vi "Day 9.vi"() -> ()   [LabVIEW 2021]
uses:
  e82450e5-71a3-46d6-8b92-650601a06453.vi
  <vilib>/Utility/file.llb/Read Delimited Spreadsheet (string).vi
  <vilib>/Comparison/Less/Less Functor/Less Functor.lvclass
panel:
  out "x-y":dbl
  out "Data":i32[][](array[numeric])
  out "Intensity Graph":i32[][](graph)
  out "Solution":i32
  in  "Input File":enum32{"example input", "input"}(radio)
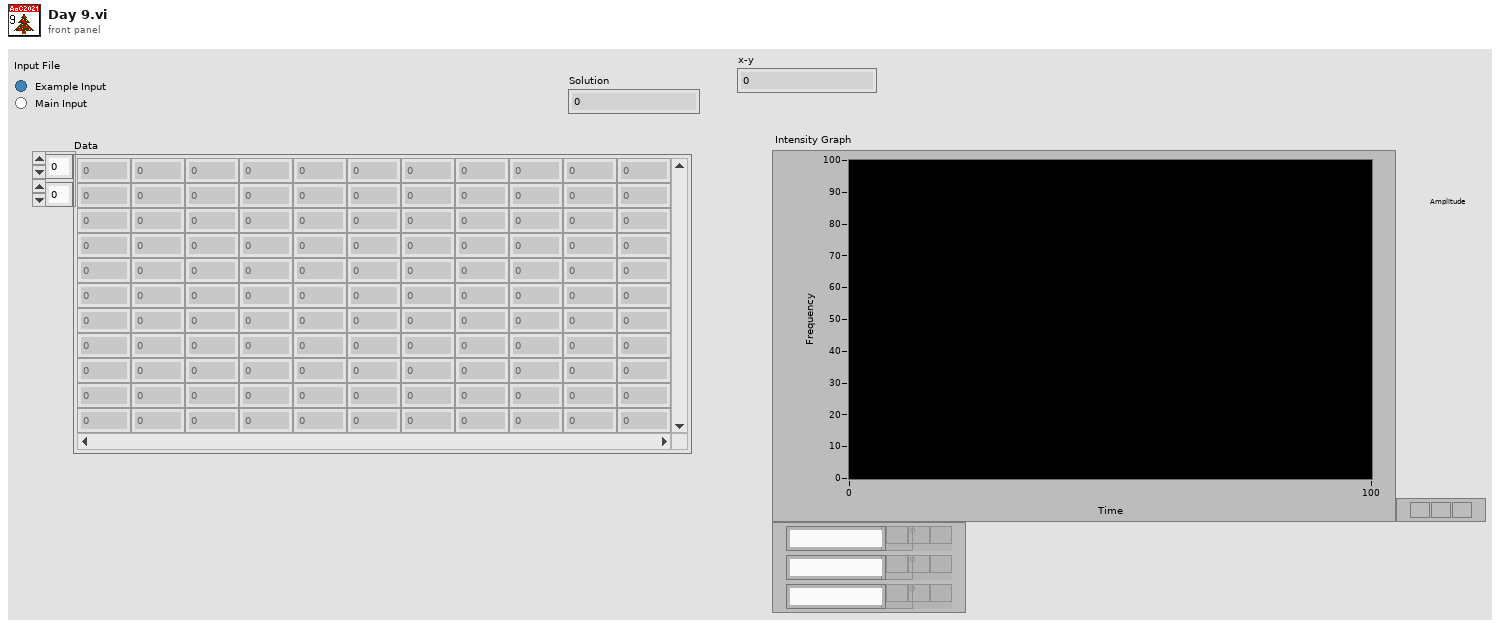
[diagram p1: front panel]
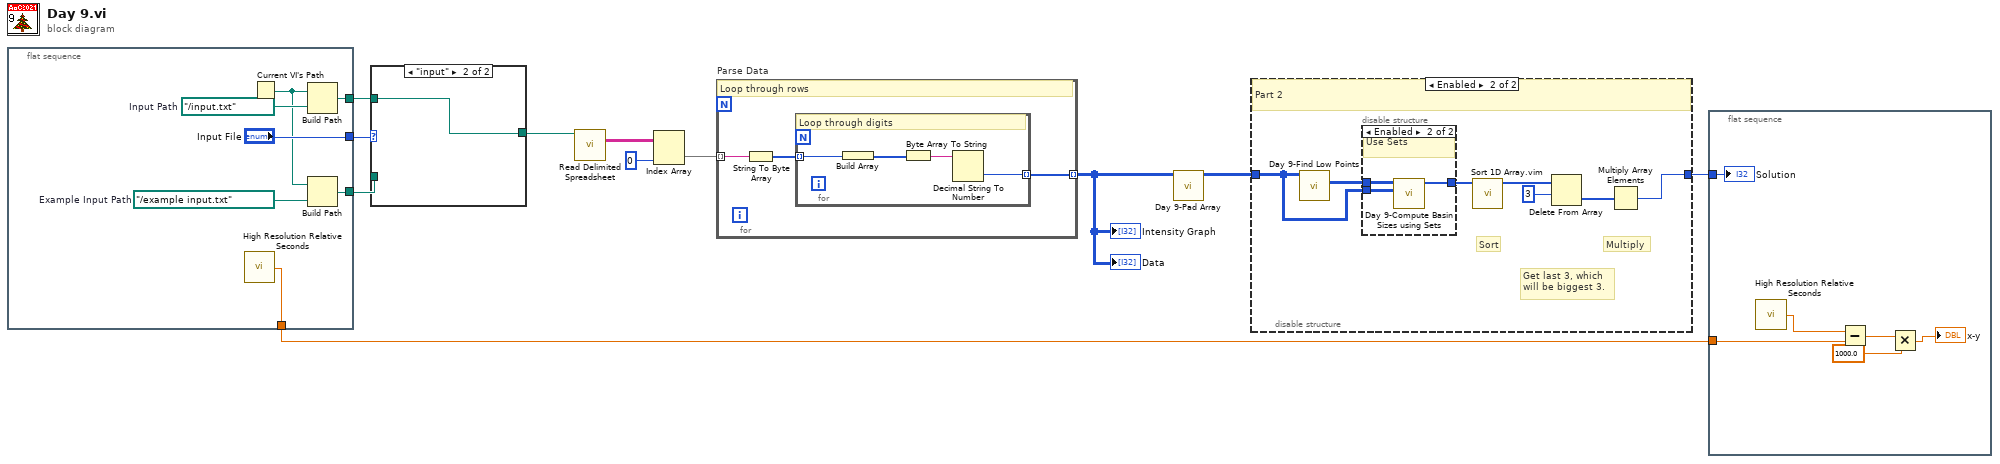
[diagram p0: block diagram]
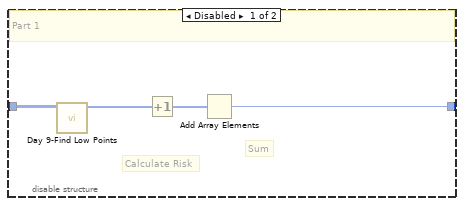
[diagram p3: hidden frame]
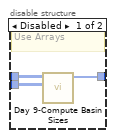
[diagram p4: hidden frame]
diagram:
  n1 = flat-sequence {
    tunnel: ["Input File"] -> w11
    tunnel: [w15] -> w10
    tunnel: [w14] -> w9
    tunnel: [w12] -> w1
    frame #0 {
      w17 = path "../example input.txt"  # Example Input Path
      w18 = path "../input.txt"  # Input Path
      n2 = call <vilib>:"High Resolution Relative Seconds.vi"() -> ("relative seconds"=w12:dbl)
      n3 = Current VI's Path() -> (path=w13:path)
      n4 = Build Path(base path=w13, name or relative path=w18) -> (appended path=w15:path)
      n5 = Build Path(base path=w13, name or relative path=w17) -> (appended path=w14:path)
    }
  }
  n6 = case shown="\"input\"" w11 {
    tunnel: w10 -> [_ w20]
    tunnel: w9 -> [w19 _]
    tunnel: [w19 w20] -> w8
    frame "example input" {
    }
    frame "input" {
    }
  }
  n7 = call-poly <vilib>:"Read Delimited Spreadsheet.vi"("file path (dialog if empty)"=w8) -> ("all rows"=w7:string[][])  [unwired: 9 in, 5 out]
  n8 = Index Array(array=w7, index (col)=0 ("disabled index (col)")) -> (element=w5:string[])  [unwired: 1 in]
  n9 = for "Parse Data" {
    tunnel: w5 -> [w23] mode=indexing
    tunnel: [w21] -> w3 mode=indexing
    # "Loop through rows"
    n10 = String To Byte Array(string=w23) -> (unsigned byte array=w22:u8[])
    n11 = for {
      tunnel: w22 -> [w27] mode=indexing
      tunnel: [w24] -> w21 mode=indexing
      # "Loop through digits"
      n12 = Build Array(w27) -> (w26:u8[])
      n13 = Byte Array To String(unsigned byte array=w26) -> (string=w25:string)
      n14 = Decimal String To Number(string=w25) -> (number=w24:i32)  [unwired: 2 in, 1 out]
    }
  }
  "Intensity Graph" <- w3
  "Data" <- w3
  n15 = call "Day 9-Pad Array.vi"("Array in"=w3) -> ("Array out"=w2:i32[][])  [unwired: 10 in]
  n16 = disable-structure shown="Enabled" {
    disable-tunnel: [w31 w34] -> w4
    disable-tunnel: w2 -> [w29 w32]
    frame Disabled {
      # "Sum"
      # "Calculate Risk"
      # "Part 1"
      n17 = call "Day 9-Find Low Points.vi"("Array in"=w29) -> ("Low Point Values"=w28:i32[])  [unwired: 9 in, 1 out]
      n18 = Increment(x=w28) -> (x+1=w30:i32[])
      n19 = Add Array Elements(numeric array=w30) -> (sum=w31:i32)
    }
    frame Enabled {
      # "Multiply"
      # "Get last 3, which will be biggest 3."
      # "Sort"
      # "Part 2"
      n20 = call "Day 9-Find Low Points.vi"("Array in"=w32) -> ("Low Point Coordinates"=w33:i32[][])  [unwired: 9 in, 1 out]
      n21 = disable-structure shown="Enabled" {
        disable-tunnel: [w41 w44] -> w38
        disable-tunnel: w33 -> [w40 w43]
        disable-tunnel: w32 -> [w39 w42]
        frame Disabled {
          # "Use Arrays"
          n22 = call "Day 9-Compute Basin Sizes.vi"("Padded Data Array in"=w39, "Low Point Coordinates"=w40) -> ("All Basin Sizes"=w41:i32[])  [unwired: 9 in]
        }
        frame Enabled {
          # "Use Sets"
          n23 = call "Day 9-Compute Basin Sizes using Sets.vi"("Padded Data Array in"=w42, "Low Point Coordinates"=w43) -> ("All Basin Sizes"=w44:i32[])  [unwired: 9 in]
        }
      }
      n24 = call "Sort 1D Array.vim"("unsorted array"=w38) -> ("sorted array"=w37:i32[])  [unwired: 10 in]
      n25 = Delete From Array(array=w37, length=3) -> (deleted portion=w35:i32[])  [unwired: 1 in, 1 out]
      n26 = Multiply Array Elements(1:w35) -> (0:w34:i32)
    }
  }
  n27 = flat-sequence {
    tunnel: w4 -> [w50]
    tunnel: w1 -> [w48]
    frame #0 {
      n28 = call <vilib>:"High Resolution Relative Seconds.vi"() -> ("relative seconds"=w49:dbl)
      n29 = Subtract(x=w49, y=w48) -> (x-y=w47:dbl)
      n30 = Multiply(x=w47, y=1000.0) -> (x*y=→"x-y":dbl)
      "Solution" <- w50
    }
  }
